vi "Close.vi"(8 "error in (no error)":errorcluster, 11 "PGJDPResult in":refnum<class "Result.lvclass">) -> (0 "error out":errorcluster)   [LabVIEW 2020, in "ORM_sqlite_jdp.lvlib" / "Result.lvclass"]
uses:
  Result.lvclass
  Result.lvclass/Result.ctl
  <vilib>/drjdpowell/SQLite Library/SQL Statement/SQL Statement.lvclass/SQL Statement.ctl
  <vilib>/Viviota/shared/ORM.lvlibp/Query Result/Query Result.lvclass
  <vilib>/drjdpowell/SQLite Library/SQL Statement/SQL Statement.lvclass
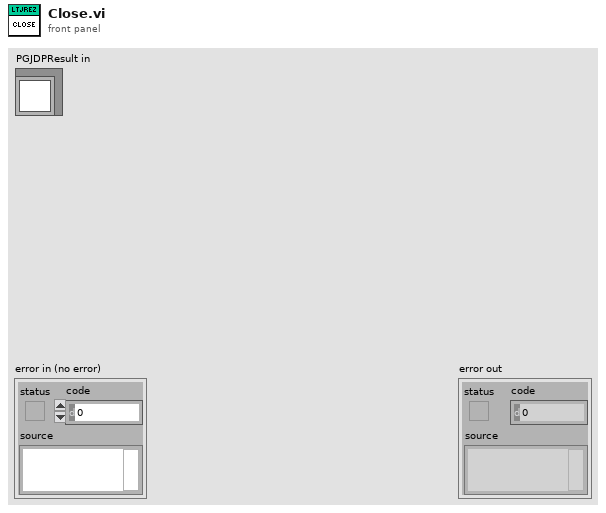
[diagram p1: front panel]
types:
  T1 = cluster{"SQL Statement":refnum<class "SQL Statement.lvclass">, "Headers":string[], "DeclaredTypes":string[]}
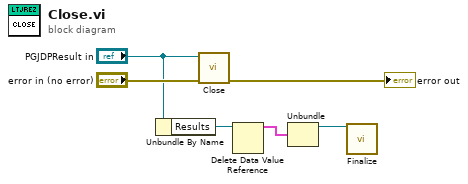
[diagram p0: block diagram]
diagram:
  n1 = Unbundle By Name("PGJDPResult in") -> ("Results"=w3:refnum<data-value>)
  n2 = call-parent "Close.vi"("error in (no error)"="error in (no error)", "Query Result in"="PGJDPResult in") -> ("error out"=→"error out":errorcluster)  [unwired: 9 in]
  n3 = Delete Data Value Reference(data value reference=w3) -> (data value=w2:T1)  [unwired: 1 in, 1 out]
  n4 = Unbundle(w2) -> ("SQL Statement"=w1:refnum<class "SQL Statement.lvclass">)  [unwired: 2 out]
  n5 = call <vilib>:"Finalize.vi"("SQL Statement in"=w1) -> ()  [unwired: 10 in, 1 out]
